vi "Get Document Reference.vi"(8 "error in (no error)":errorcluster, 11 "ooDocument in":refnum<class "ooDocument.lvclass">) -> (0 "error out":errorcluster, 1 "Document":refnum<k24>, 3 "ooDocument out":refnum<class "ooDocument.lvclass">)   [LabVIEW 2009, in "ooDocument.lvclass"]
uses:
  ooDocument.lvclass
  C:/Projets/LAVAG/OpenOfficeRGT/AODL/DLLs/AODL.dll
  ooDocument.lvclass/ooDocument.ctl
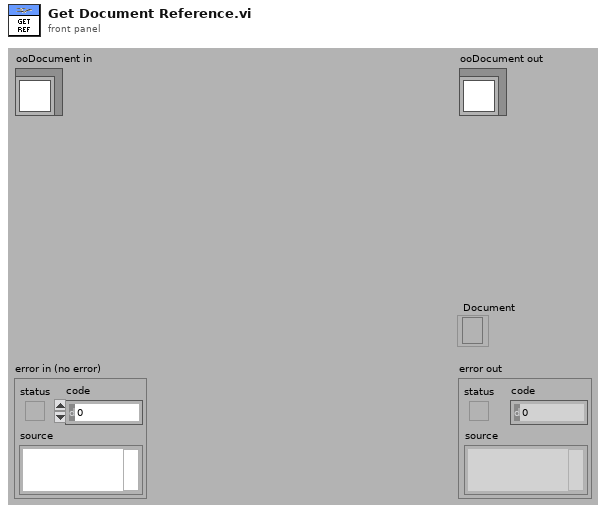
[diagram p1: front panel]
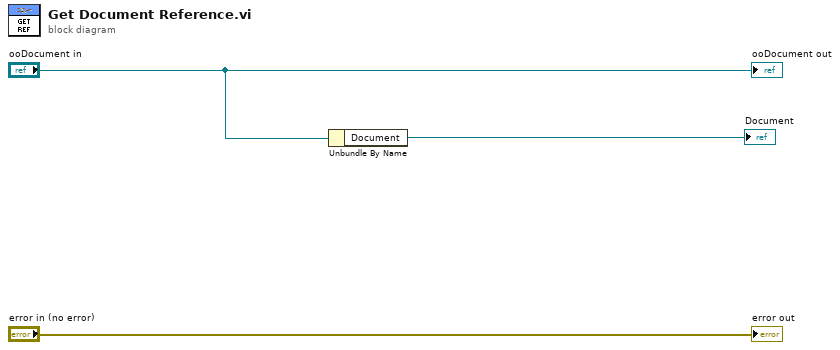
[diagram p0: block diagram]
diagram:
  n1 = Unbundle By Name("ooDocument in") -> ("Document"=→"Document":refnum<k24>)
  "error out" <- "error in (no error)"
  "ooDocument out" <- "ooDocument in"
